vi "Facade.vi"(0 "Data In":T4, 2 "Display State In":T2, 3 "Container State":T3) -> (6 "Data Out":T4, 7 "Display State Out":T2, 8 "Action":T1)   [LabVIEW 2012, in "Hide Panel.xctl"]
uses:
  Hide Panel.xctl
  Data.ctl
  <vilib>/_xctls/Container State.ctl
  State.ctl
  <vilib>/_xctls/Action.ctl
  <vilib>/_xctls/XControlSupport.lvlib
types:
  T1 = typedef "XControlSupport.lvlib/Action.ctl" = cluster{"Data Changed?":bool, "State Changed?":bool, "Action Name":string}
  T2 = typedef "Hide Panel.xctl/State.ctl" = cluster{"VI Refnum":refnum<vi>, "State":bool}
  T3 = typedef "XControlSupport.lvlib/Container State.ctl" = cluster{"Indicator?":bool, "Run Mode?":bool, " Refnum":refnum<vi>}
  T4 = typedef "Hide Panel.xctl/Data.ctl" = bool
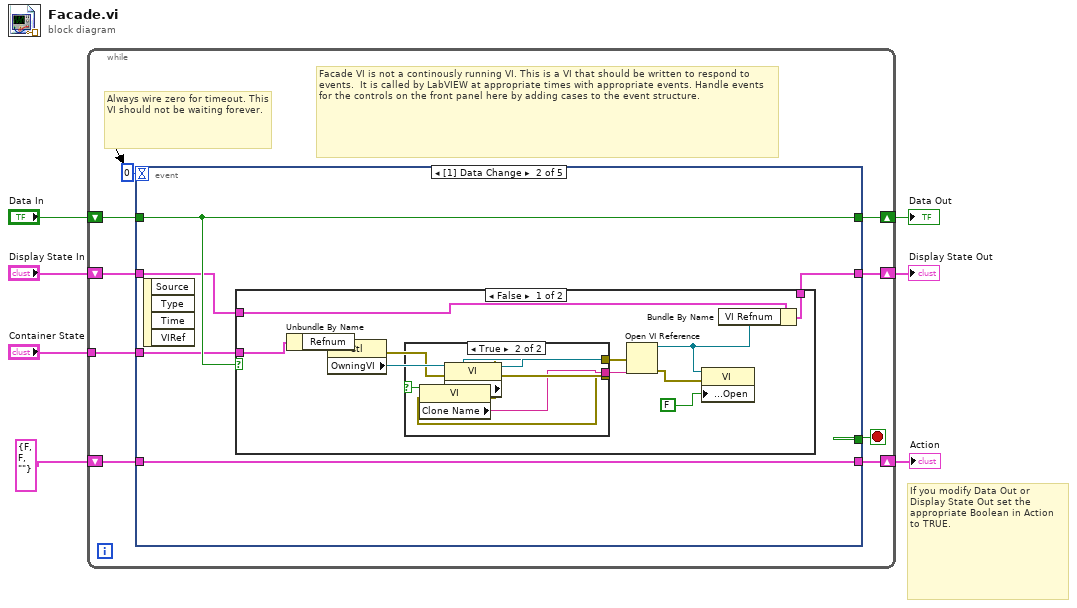
[diagram p0: block diagram]
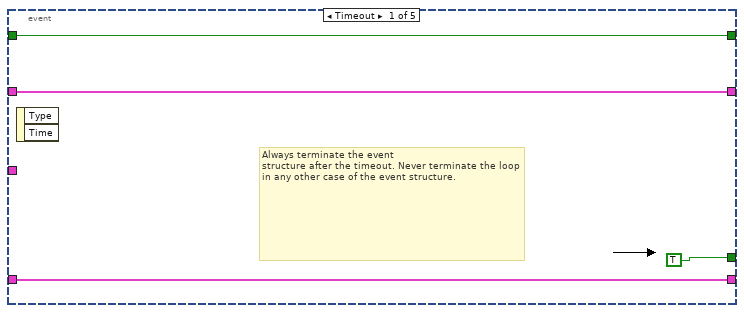
[diagram p2: hidden frame]
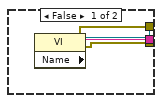
[diagram p3: hidden frame]
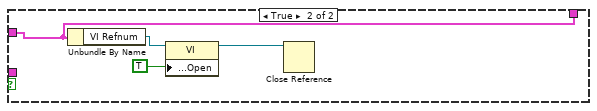
[diagram p4: hidden frame]
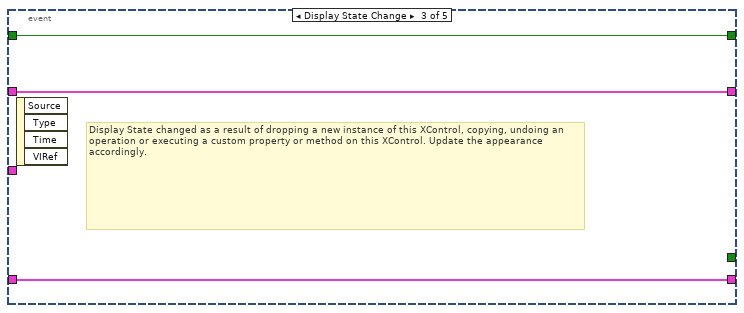
[diagram p5: hidden frame]
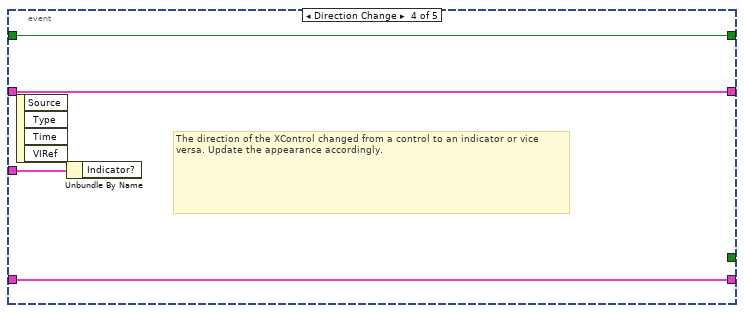
[diagram p6: hidden frame]
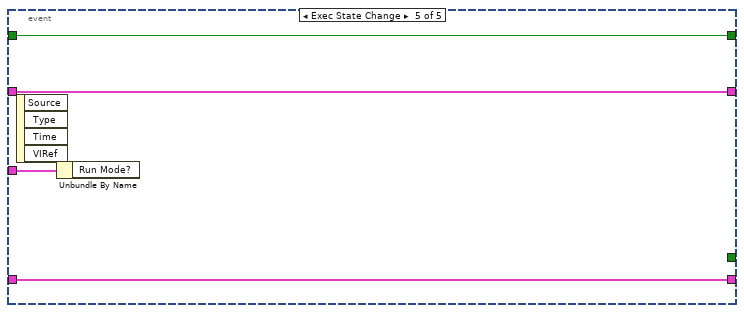
[diagram p7: hidden frame]
diagram:
  # "If you modify Data Out or\nDisplay State Out set the\nappropriate Boolean in Action\nto TRUE."
  n1 = while {
    shift-right: [w15] -> w4
    shift-left: "Display State In" -> [w16]
    tunnel: "Container State" -> [w12]
    shift-right: [w10] -> w7
    shift-left: "Data In" -> [w11]
    shift-right: [w8] -> w2
    shift-left: T1 {"Data Changed?"=FALSE, "State Changed?"=FALSE, "Action Name"=""} ("Action") -> [w9]
    stop <- w14 stop-if-true
    # "Facade VI is not a continously running VI. This is a VI that should be written to respond to events.  It is called by LabVIEW at appropriate times with appropriate events. Handle events for the controls on the front panel here by adding cases to the event structure."
    # "Always wire zero for timeout. This\nVI should not be waiting forever."
    n2 = event shown="[1] Data Change" {
      selector: _ -> [_ _ _ _ _]
      dyn-events: _ -> [_ _ _ _ _]
      timeout: 0 -> [_ _ _ _ _]
      tunnel: w16 -> [w18 w22 w54 w57 w60]
      tunnel: [w18 w21 w54 w57 w60] -> w15
      tunnel: [TRUE _ _ _ _] -> w14
      tunnel: w12 -> [_ w23 _ w58 w62]
      tunnel: w11 -> [w17 w24 w53 w56 w59]
      tunnel: [w17 w24 w53 w56 w59] -> w10
      tunnel: [w19 w25 w52 w55 w61] -> w8
      tunnel: w9 -> [w19 w25 w52 w55 w61]
      event Timeout {
        # "Always terminate the event\nstructure after the timeout. Never terminate the loop in any other case of the event structure."
        n3 = event-data() -> ()  [unwired: 3 out]
      }
      event Data Change {
        n4 = event-data() -> ()  [unwired: 5 out]
        n5 = case shown="False" w24 {
          tunnel: w23 -> [w31 _]
          tunnel: w22 -> [w30 w48]
          tunnel: [w29 w48] -> w21
          frame False {
            n6 = Unbundle By Name(w31) -> ("Refnum"=w39:refnum<vi>)
            n7 = property class="Ctl"(reference=w39) -> (error out=w33:errorcluster, "OwningVI"=w38:refnum<vi>)  [unwired: 1 in, 1 out]
            n8 = property class="VI"(reference=w38, error in=w33) -> (reference out=w35:refnum<vi>, error out=w36:errorcluster, "IsCloneVI"=w37:bool)
            n9 = case shown="True" w37 {
              tunnel: w36 -> [w42 w47]
              tunnel: w35 -> [w43 w46]
              tunnel: [w40 w45] -> w34
              tunnel: [w41 w44] -> w32
              frame False {
                n10 = property class="VI"(reference=w43, error in=w42) -> (error out=w41:errorcluster, "Name"=w40:string)  [unwired: 1 out]
              }
              frame True {
                n11 = property class="VI"(reference=w46, error in=w47) -> (error out=w44:errorcluster, "Clone Name"=w45:string)  [unwired: 1 out]
              }
            }
            n12 = Open VI Reference(vi path=w34, error in (no error)=w32) -> (vi reference=w28:refnum<vi>, error out=w27:errorcluster)  [unwired: 1 in, 3 out]
            n13 = property class="VI"(reference=w28, error in=w27, "Front Panel.Open"=FALSE) -> ()  [unwired: 2 out]
            n14 = Bundle By Name(cluster=w30, "VI Refnum"=w28) -> (w29:T2)
          }
          frame True {
            n15 = Unbundle By Name(w48) -> ("VI Refnum"=w51:refnum<vi>)
            n16 = property class="VI"(reference=w51, "Front Panel.Open"=TRUE ("Front Panel Window:Open")) -> (reference out=w49:refnum<vi>)  [unwired: 1 in, 1 out]
            n17 = Close Reference(reference=w49) -> ()  [unwired: 1 in, 1 out]
          }
        }
      }
      event Display State Change {
        # "Display State changed as a result of dropping a new instance of this XControl, copying, undoing an operation or executing a custom property or method on this XControl. Update the appearance accordingly."
        n18 = event-data() -> ()  [unwired: 5 out]
      }
      event Direction Change {
        # "The direction of the XControl changed from a control to an indicator or vice versa. Update the appearance accordingly."
        n19 = event-data() -> ()  [unwired: 5 out]
        n20 = Unbundle By Name(w58) -> ()  [unwired: 1 out]
      }
      event Exec State Change {
        n21 = event-data() -> ()  [unwired: 5 out]
        n22 = Unbundle By Name(w62) -> ()  [unwired: 1 out]
      }
    }
  }
  "Display State Out" <- w4
  "Data Out" <- w7
  "Action" <- w2
